vi "MQTT Subscriptions - Handle Subscribe.vi"(0 "MQTT ref in":T2, 5 "Packet ID":u16, 7 "Subscriptions":cluster{"MQTT Topic Filter":string, "QoS":T1}[](array[cluster]), 11 "error in":errorcluster) -> (4 "MQTT ref out":T2, 15 "error out":errorcluster)   [LabVIEW 2019, in "KoRE-MQTT.lvlib"]
doc: "Copyright (c) 2025 KoRElibs.com\nSPDX-License-Identifier: EUPL-1.2\n\nThis VI is licensed under the European Union Public License (EUPL) Version 1.2. You may use this VI unmodified in proprietary works. If you distribute a modified version of this file, the modified file must be released under the EUPL-1.2. Full license: https://joinup.ec.europa.eu/asset/eupl/eupl/1.2/"
uses:
  KoRE-MQTT.lvlib
  Public/TypeDefs/MQTT Client Session.ctl
  Public/TypeDefs/MQTT QoS Level.ctl
  TypeDefs/MQTT Client Session - Data Value Reference.ctl
  Public/TypeDefs/MQTT Client Session - Data.ctl
  Public/TypeDefs/MQTT Property - Will.ctl
  Public/TypeDefs/MQTT Property - CONNECT.ctl
  TypeDefs/MQTT Subscription - Info.ctl
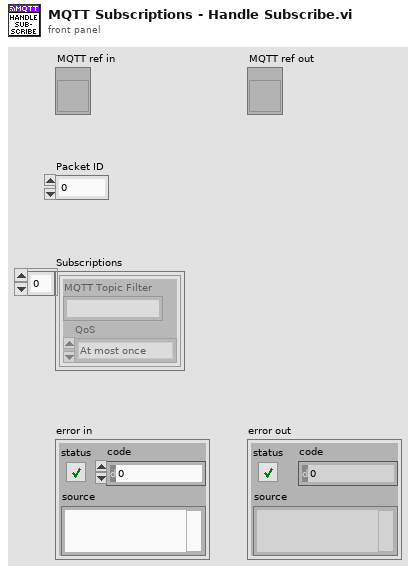
[diagram p1: front panel]
types:
  T1 = typedef "KoRE-MQTT.lvlib/MQTT QoS Level.ctl" = enum8{"At most once", "At least once", "Exactly once"}
  T2 = typedef "KoRE-MQTT.lvlib/MQTT Client Session.ctl" = refnum<vi>
  T3 = typedef "KoRE-MQTT.lvlib/MQTT Client Session - Data Value Reference.ctl" = refnum<data-value>
  T4 = typedef "KoRE-MQTT.lvlib/MQTT Subscription - Info.ctl" = cluster{"Packet Id":u16, "Index":u16, "Identifier":u32, "QoS":u8, "Topic Filter":string, "Reason Code":u8, "Reason String":string, "Granted":bool}
  T5 = typedef "KoRE-MQTT.lvlib/MQTT Client Session - Data.ctl" = cluster{"TCP ref":refnum<k5>, "Next Packet Id":u16, "Version":u8, "Host":string, "Port":u16, "Ping Delta":u32, "Username":string, "Password":string, "Will QoS":u8, "Will Retain":bool, "Will Topic":string, "Will Payload":string, "TCP Timeout":i32, "Semaphore":T6, "In-Flight Messages":variant, "Close":bool, "Last Send":u32, "Keep Alive":u16, "Last Ping RTT":u32, "Last Ping":u32, "Will Properties":T7[], "Session Expiry Interval":u32, "Maximum QoS":u8, "Retain Available":bool, "Server Maximum Packet Size":u32, "Client Identifier":string, "Server Topic Alias Maximum":u16, "Wildcard Subscription Available":bool, "Subscription Identifier Available":bool, "Shared Subscription Available":bool, "Connect Properties":T8[], "Client Maximum Packet Size":u32, "Client Topic Alias Maximum":u16, "Server Receive Maximum":u16, "Client Receive Maximum":u16, "TLS cfg":refnum<k36>, "Subscriptions":T4[]}
  T6 = typedef "Semaphore RefNum" = refnum<k1>
  T7 = typedef "KoRE-MQTT.lvlib/MQTT Property - Will.ctl" = cluster{"Property":u8, "Value":string}
  T8 = typedef "KoRE-MQTT.lvlib/MQTT Property - CONNECT.ctl" = cluster{"Property":u8, "Value":string}
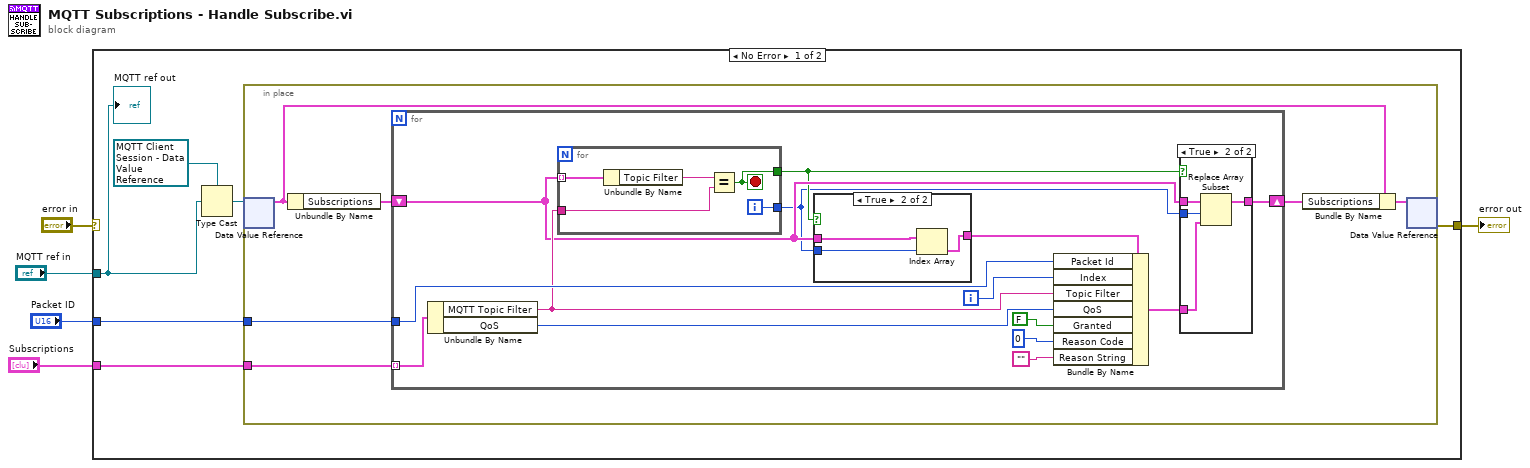
[diagram p0: block diagram]
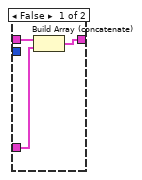
[diagram p2: hidden frame]
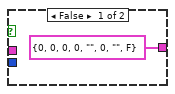
[diagram p3: hidden frame]
diagram:
  n1 = case shown="No Error" "error in" {
    selector: "error in" -> [_ w48]
    tunnel: "Packet ID" -> [w11 _]
    tunnel: "MQTT ref in" -> [w9 _]
    tunnel: "Subscriptions" -> [w7 _]
    tunnel: [w6 w48] -> w2
    frame No Error {
      n2 = Type Cast(type=T3 refnum ("data value reference"), x=w9) -> (*(type *) &x=w10:T3)
      n3 = in-place {
        in-place-border: w11 -> [w17]
        in-place-border: w7 -> [w12]
        n4 = in-place-dvr #1(w10) -> (w13:T5)  [unwired: 1 out]
        n5 = Unbundle By Name(w13) -> ("Subscriptions"=w16:T4[])
        n6 = for {
          tunnel: w17 -> [w30]
          shift-right: [w23] -> w15
          shift-left: w16 -> [w25]
          tunnel: w12 -> [w31] mode=indexing
          i -> [w29]
          n7 = Unbundle By Name(w31) -> ("MQTT Topic Filter"=w27:string, "QoS"=w28:T1)
          n8 = for {
            tunnel: w25 -> [w47] mode=indexing
            tunnel: w27 -> [w45]
            tunnel: [w44] -> w22
            tunnel: [w43] -> w21
            i -> [w43]
            stop <- w44 stop-if-true
            n9 = Unbundle By Name(w47) -> ("Topic Filter"=w46:string)
            n10 = Equal?(x=w46, y=w45) -> (x = y?=w44:bool)
          }
          n11 = case shown="True" w22 {
            tunnel: [T4 {"Packet Id"=0, "Index"=0, "Identifier"=0, "QoS"=0, "Topic Filter"="", "Reason Code"=0, "Reason String"="", "Granted"=FALSE} ("Subscription Info") w40] -> w26
            tunnel: w25 -> [_ w42]
            tunnel: w21 -> [_ w41]
            frame False {
            }
            frame True {
              n12 = Index Array(array=w42, index=w41) -> (element=w40:T4)
            }
          }
          n13 = Bundle By Name(cluster=w26, "Packet Id"=w30, "Index"=w29, "Topic Filter"=w27, "QoS"=w28, "Granted"=FALSE, "Reason Code"=u8 0, "Reason String"="") -> (w24:T4)
          n14 = case shown="True" w22 {
            tunnel: w25 -> [w34 w38]
            tunnel: w24 -> [w33 w36]
            tunnel: [w32 w35] -> w23
            tunnel: w21 -> [_ w37]
            frame False {
              n15 = Build Array (concatenate)(w34, w33) -> (w32:T4[])
            }
            frame True {
              n16 = Replace Array Subset(array=w38, new element=w36, index=w37) -> (w35:T4[])
            }
          }
        }
        n17 = Bundle By Name(cluster=w13, "Subscriptions"=w15) -> (w14:T5)
        n18 = in-place-dvr #1(w14) -> (w6:errorcluster)  [unwired: 1 out]
      }
      "MQTT ref out" <- w9
    }
    frame Error {
    }
  }
  "error out" <- w2
